vi "measure BT Dwell Time.vi"(8 "error in (no error)":errorcluster, 10 "Threshold Level":dbl, 11 "SA Measurement in":refnum<class "SA Measurement.lvclass">) -> (0 "error out":errorcluster, 3 "SA Measurement out":refnum<class "SA Measurement.lvclass">)   [LabVIEW 2023, in "Spectrum Analyzer.lvlib" / "SA Measurement.lvclass"]
uses:
  SA Measurement.lvclass
  SA Measurement.lvclass/SA Measurement.ctl
  TYPE DEFINITION/Keysight 9020A/TYPE Measurement Preset.ctl
  Spectrum Analyzer.lvlib
  TYPE DEFINITION/TYPE RBW and VBW Select.ctl
  Interface_Spectrum/Interface_Spectrum.lvclass
  <vilib>/Utility/file.llb/Read Delimited Spreadsheet (string).vi
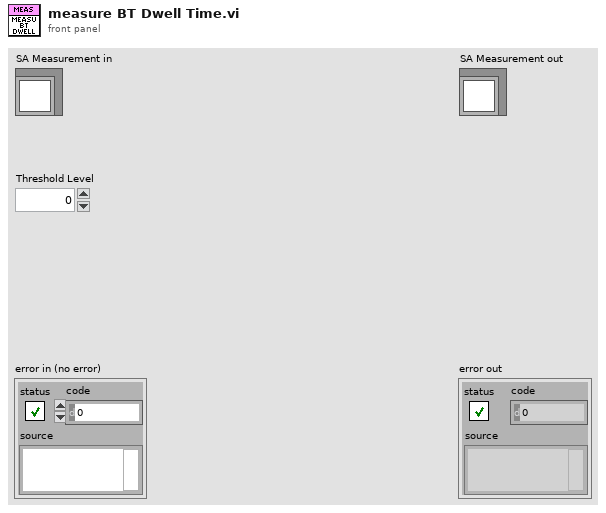
[diagram p1: front panel]
types:
  T1 = typedef "Spectrum Analyzer.lvlib/TYPE RBW and VBW Select.ctl" = enum16{"Res BW", "Video BW"}
  T2 = typedef "Spectrum Analyzer.lvlib/TYPE Measurement Preset.ctl" = enum16{"Sweep SA Mode", "Channel Power", "Occupied BW", "ACP", "Spurious Emission", "Spurious Emission Mask", "Burst Power (Transmit Power)"}
  T3 = typedef "Spectrum Analyzer.lvlib/TYPE Reference Level and Atten Param.ctl" = cluster{"Reference Level":dbl, "Atten":i32, "Atten Auto?":bool, "Reference Level Offset":dbl}
  T4 = typedef "Spectrum Analyzer.lvlib/TYPE Display Trace Mode Select.ctl" = enum16{"Clear Write", "Max Hold", "Min Hold", "Average", "View"}
  T5 = typedef "Spectrum Analyzer.lvlib/TYPE Detect Mode Select.ctl" = enum16{"Det Auto (Normal)", "Auto Peak", "Positive Peak", "Negative Peak", "Sample", "RMS", "Average", "Quasipeak", "CISPR Average", "RMS Average"}
  T6 = cluster{"Trace Mode":T4, "Detector Type":T5, "Detect Auto?":bool}[]
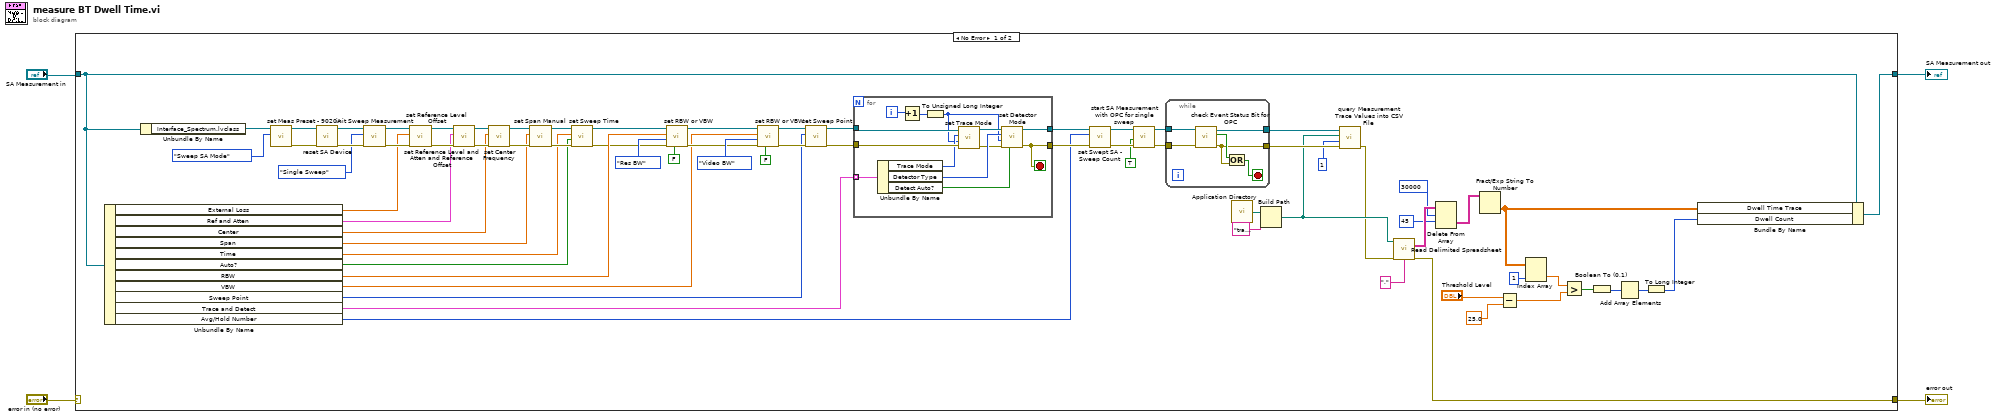
[diagram p0: block diagram]
diagram:
  n1 = case shown="No Error" "error in (no error)" {
    selector: "error in (no error)" -> [_ w97]
    tunnel: [w5 w97] -> w1
    tunnel: [w40 w96] -> w2
    tunnel: "SA Measurement in" -> [w41 w96]
    frame No Error {
      n2 = Unbundle By Name(w41) -> ("External Loss"=w65:dbl, "Ref and Atten"=w64:T3, "Center"=w37:dbl, "Span"=w34:dbl, "Time"=w31:dbl, "Auto?"=w30:bool, "RBW"=w57:dbl, "VBW"=w56:dbl, "Sweep Point"=w53:u32, "Trace and Detect"=w50:T6, "Avg/Hold Number"=w47:u32)
      n3 = Unbundle By Name(w41) -> ("Interface_Spectrum.lvclass"=w76:refnum<class "Interface_Spectrum.lvclass">)
      n4 = call-dynamic "set Meas Preset - 9020A.vi"("Measurement Preset"=TYPE_Measurement_Preset."Sweep SA Mode", "Interface_Spectrum in"=w76) -> ("error out"=w73:errorcluster, "Interface_Spectrum out"=w74:refnum<class "Interface_Spectrum.lvclass">)  [unwired: 8 in]
      n5 = call-dynamic "reset SA Device.vi"("error in (no error)"=w73, "Interface_Spectrum in"=w74) -> ("error out"=w71:errorcluster, "Interface_Spectrum out"=w72:refnum<class "Interface_Spectrum.lvclass">)  [unwired: 8 in]
      n6 = call-dynamic "init Sweep Measurement.vi"("error in (no error)"=w71, "Sweep Measurement Mode"=enum16{"Single Sweep", "Continuous Sweep"}."Single Sweep", "Interface_Spectrum in"=w72) -> ("error out"=w68:errorcluster, "Interface_Spectrum out"=w69:refnum<class "Interface_Spectrum.lvclass">)  [unwired: 7 in]
      n7 = call-dynamic "set Reference Level Offset.vi"("error in (no error)"=w68, "Reference Level Offset"=w65, "Interface_Spectrum in"=w69) -> ("error out"=w66:errorcluster, "Interface_Spectrum out"=w67:refnum<class "Interface_Spectrum.lvclass">)  [unwired: 7 in]
      n8 = call-dynamic "set Reference Level and Atten and Reference Offset.vi"("error in (no error)"=w66, "Reference Level, Atten, Reference Offset"=w64, "Interface_Spectrum in"=w67) -> ("error out"=w38:errorcluster, "Interface_Spectrum out"=w39:refnum<class "Interface_Spectrum.lvclass">)  [unwired: 7 in]
      n9 = call-dynamic "set Center Frequency.vi"("error in (no error)"=w38, "Center Frequency (Hz)"=w37, "Interface_Spectrum in"=w39) -> ("error out"=w35:errorcluster, "Interface_Spectrum out"=w36:refnum<class "Interface_Spectrum.lvclass">)  [unwired: 7 in]
      n10 = call-dynamic "set Span Manual.vi"("error in (no error)"=w35, "Span (Hz)"=w34, "Interface_Spectrum in"=w36) -> ("error out"=w32:errorcluster, "Interface_Spectrum out"=w33:refnum<class "Interface_Spectrum.lvclass">)  [unwired: 7 in]
      n11 = call-dynamic "set Sweep Time.vi"("error in (no error)"=w32, "Sweep Time Auto?"=w30, "Sweep Time(sec)"=w31, "Interface_Spectrum in"=w33) -> ("error out"=w28:errorcluster, "Interface_Spectrum out"=w29:refnum<class "Interface_Spectrum.lvclass">)  [unwired: 6 in]
      n12 = call-dynamic "set RBW or VBW.vi"("BW Auto?"=FALSE, "error in (no error)"=w28, "BW Type"=TYPE_RBW_and_VBW_Select."Res BW", "BW Value (Hz)"=w57, "Interface_Spectrum in"=w29) -> ("error out"=w58:errorcluster, "Interface_Spectrum out"=w59:refnum<class "Interface_Spectrum.lvclass">)  [unwired: 5 in]
      n13 = call-dynamic "set RBW or VBW.vi"("BW Auto?"=FALSE, "error in (no error)"=w58, "BW Type"=TYPE_RBW_and_VBW_Select."Video BW", "BW Value (Hz)"=w56, "Interface_Spectrum in"=w59) -> ("error out"=w54:errorcluster, "Interface_Spectrum out"=w55:refnum<class "Interface_Spectrum.lvclass">)  [unwired: 5 in]
      n14 = call-dynamic "set Sweep Point.vi"("error in (no error)"=w54, "Sweep Point"=w53, "Interface_Spectrum in"=w55) -> ("error out"=w51:errorcluster, "Interface_Spectrum out"=w52:refnum<class "Interface_Spectrum.lvclass">)  [unwired: 7 in]
      n15 = for {
        tunnel: w52 -> [w94]
        tunnel: w51 -> [w93]
        tunnel: w50 -> [w95] mode=indexing
        tunnel: [w83] -> w48
        tunnel: [w84] -> w49
        i -> [w92]
        stop <- w83 stop-if-true
        n16 = Unbundle By Name(w95) -> ("Trace Mode"=w90:T4, "Detector Type"=w88:T5, "Detect Auto?"=w85:bool)
        n17 = Increment(x=w92) -> (x+1=w91:i32)
        n18 = To Unsigned Long Integer(number=w91) -> (unsigned 32bit integer=w86:u32)
        n19 = call-dynamic "set Trace Mode.vi"("error in (no error)"=w93, "Trace Index"=w86, "Trace Mode"=w90, "Interface_Spectrum in"=w94) -> ("error out"=w87:errorcluster, "Interface_Spectrum out"=w89:refnum<class "Interface_Spectrum.lvclass">)  [unwired: 6 in]
        n20 = call-dynamic "set Detector Mode.vi"("Detect Auto?"=w85, "error in (no error)"=w87, "Trace Index"=w86, "Detector Type"=w88, "Interface_Spectrum in"=w89) -> ("error out"=w83:errorcluster, "Interface_Spectrum out"=w84:refnum<class "Interface_Spectrum.lvclass">)  [unwired: 5 in]
      }
      n21 = call-dynamic "set Swept SA - Sweep Count.vi"("error in (no error)"=w48, "Sweep Count"=w47, "Interface_Spectrum in"=w49) -> ("error out"=w45:errorcluster, "Interface_Spectrum out"=w46:refnum<class "Interface_Spectrum.lvclass">)  [unwired: 7 in]
      n22 = call-dynamic "start SA Measurement with OPC for single sweep.vi"("error in (no error)"=w45, "with OPC?"=TRUE, "Interface_Spectrum in"=w46) -> ("error out"=w42:errorcluster, "Interface_Spectrum out"=w43:refnum<class "Interface_Spectrum.lvclass">)  [unwired: 7 in]
      n23 = while {
        tunnel: w43 -> [w82]
        tunnel: w42 -> [w81]
        tunnel: [w78] -> w24
        tunnel: [w77] -> w25
        stop <- w79 stop-if-true
        n24 = call-dynamic "check Event Status Bit for OPC.vi"("error in (no error)"=w81, "Interface_Spectrum in"=w82) -> ("error out"=w78:errorcluster, "OPC Bit Changed?"=w80:bool, "Interface_Spectrum out"=w77:refnum<class "Interface_Spectrum.lvclass">)  [unwired: 7 in]
        n25 = Or(x=w80, y=w78) -> (x .or. y?=w79:bool)
      }
      n26 = call <vilib>:"Application Directory.vi"() -> ("Application Directory"=w27:path)
      n27 = Build Path(base path=w27, name or relative path="traceRawdata.csv") -> (appended path=w17:path)
      n28 = call-dynamic "query Measurement Trace Values into CSV File.vi"("error in (no error)"=w24, "Trace Index"=1, "Path"=w17, "Interface_Spectrum in"=w25) -> ("error out"=w16:errorcluster)  [unwired: 6 in, 1 out]
      n29 = call-poly <vilib>:"Read Delimited Spreadsheet.vi"("file path (dialog if empty)"=w17, "error in (no error)"=w16, "delimiter (\\t)"="," ("delimiter (\\t)")) -> ("all rows"=w21:string[][], "error out"=w5:errorcluster)  [unwired: 7 in, 4 out]
      n30 = Delete From Array(array=w21, length=30000, index (row)=45) -> (deleted portion=w18:string[][])  [unwired: 1 in, 1 out]
      n31 = Fract/Exp String To Number(string=w18) -> (number=w6:dbl[][])  [unwired: 3 in, 1 out]
      n32 = Subtract(x="Threshold Level", y=25.0) -> (x-y=w8:dbl)
      n33 = Index Array(array=w6, index (col)=1 ("disabled index (col)")) -> (element=w9:dbl[])  [unwired: 1 in]
      n34 = Greater?(x=w9, y=w8) -> (0:w12:bool[])
      n35 = Boolean To (0,1)(Boolean=w12) -> (0, 1=w11:i16[])
      n36 = Add Array Elements(numeric array=w11) -> (sum=w10:i16)
      n37 = To Long Integer(number=w10) -> (32bit integer=w7:i32)
      n38 = Bundle By Name(cluster=w41, "Dwell Time Trace"=w6, "Dwell Count"=w7) -> (w40:refnum<class "SA Measurement.lvclass">)
    }
    frame Error {
    }
  }
  "error out" <- w1
  "SA Measurement out" <- w2
